vi "UpdateFeedCache.vi"(8 "error in (no error)":errorcluster, 9 "feed GUID":string, 10 "feed url":string) -> (0 "error out":errorcluster)   [LabVIEW 2023, in "GettingStartedWindow.lvlib" / "Feed_link.lvclass"]
uses:
  <resource>/modes/FRC/GSW/Classes/Feed_link/Feed_link.lvclass
  <resource>/modes/FRC/GSW/Globals.vi
  <vilib>/NI_RSS/Feed/Feed.lvclass
  <resource>/modes/FRC/GSW/GettingStartedWindow.lvlib
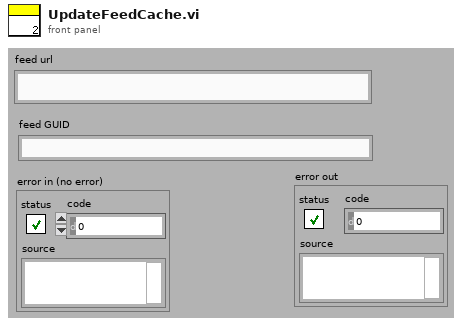
[diagram p1: front panel]
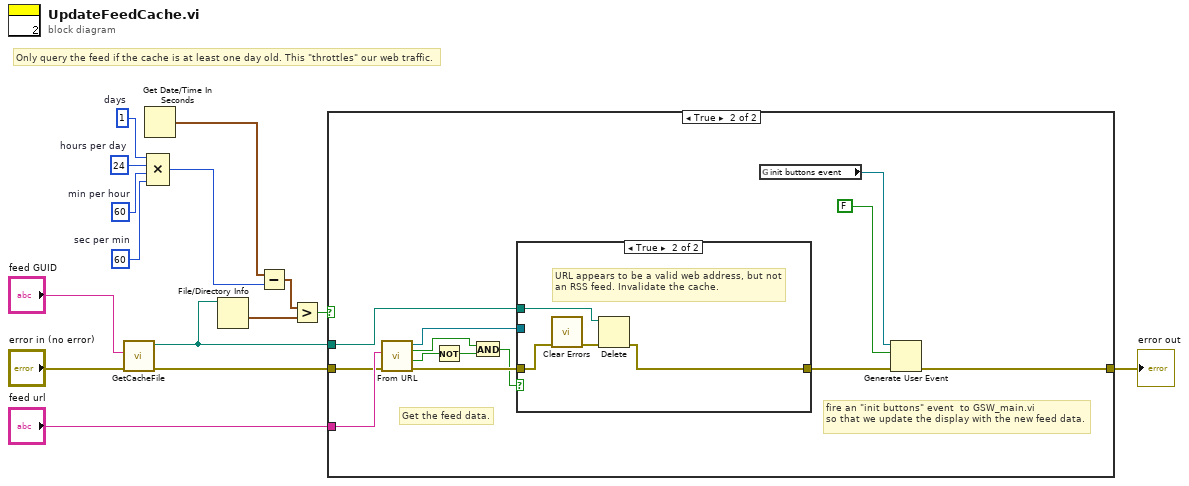
[diagram p0: block diagram]
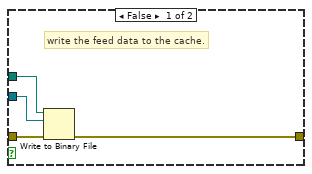
[diagram p3: hidden frame]
diagram:
  w3 = 1  # days
  w5 = 60  # sec per min
  w6 = 60  # min per hour
  w7 = 24  # hours per day
  # "Only query the feed if the cache is at least one day old. This \"throttles\" our web traffic."
  n1 = call <resource>:"GetCacheFile.vi"("error in (no error)"="error in (no error)", "feed GUID"="feed GUID") -> ("error out"=w12:errorcluster, "cache file"=w2:path)  [unwired: 8 out]
  n2 = Get Date/Time In Seconds() -> (seconds since 1Jan1904=w10:timestamp)
  n3 = Compound Arithmetic op=MULTIPLY(w3, w7, w6, w5) -> (w4:i32)
  n4 = File/Directory Info(path=w2) -> (last mod=w9:timestamp)  [unwired: 1 in, 6 out]
  n5 = Subtract(x=w10, y=w4) -> (x-y=w8:timestamp)
  n6 = Greater?(x=w8, y=w9) -> (0:w1:bool)
  n7 = case shown="True" w1 {
    tunnel: "feed url" -> [_ w29]
    tunnel: w2 -> [_ w28]
    tunnel: w12 -> [w16 w25]
    tunnel: [w16 w17] -> w11
    frame False {
    }
    frame True {
      # "fire an \"init buttons\" event  to GSW_main.vi\nso that we update the display with the new feed data."
      # "Get the feed data."
      n8 = call <vilib>:"From URL.vi"("error in (no error)"=w25, "Feed URL"=w29) -> ("error out"=w26:errorcluster, "feed valid?"=w23:bool, "url valid?"=w24:bool, "Feed out"=w27:refnum<class "Feed.lvclass">)  [unwired: 6 out]
      n9 = Not(x=w23) -> (.not. x?=w22:bool)
      n10 = And(x=w24, y=w22) -> (x .and. y?=w21:bool)
      n11 = case shown="True" w21 {
        tunnel: [w30 w34] -> w18
        tunnel: w28 -> [w33 w37]
        tunnel: w27 -> [w32 _]
        tunnel: w26 -> [w31 w36]
        frame False {
          # "write the feed data to the cache."
          n12 = Write to Binary File(file (use dialog)=w33, data=w32, error in=w31) -> (error out=w30:errorcluster)  [unwired: 5 out]
        }
        frame True {
          # "URL appears to be a valid web address, but not\nan RSS feed. Invalidate the cache."
          n13 = call <vilib>:"Clear Errors.vi"("error in (no error)"=w36) -> ("error out"=w35:errorcluster)  [unwired: 1 in, 5 out]
          n14 = Delete(path (use dialog)=w37, error in=w35) -> (error out=w34:errorcluster)  [unwired: 5 out]
        }
      }
      n15 = global read "Globals.vi" "init buttons event"() -> (w19:refnum<user-event>)
      n16 = Generate User Event(user event=w19, event data cluster=FALSE ("event data"), error in=w18) -> (error out=w17:errorcluster)  [unwired: 1 in, 1 out]
    }
  }
  "error out" <- w11
